vi "PicoScope4000aExampleBlock.vi"() -> ()   [LabVIEW 2010]
doc: "This example demonstrates how to use the PicoScope Labview library to collect data using block mode."
uses:
  shared/PicoBuffers.ctl
  shared/Buffer and Transfer Settings.ctl
  shared/Acquisition Settings.ctl
  PicoScope4000aLib/PicoScope4000aAnalogChannelSettings.ctl
panel:
  in  "roundFaster":bool=TRUE
  in  "Write to TDMS":bool
  in  "Channel B Settings":T1={"Enabled"=FALSE, "Coupling"=1, "Range"=6, "Analogue Offset"=0.0, "Bandwidth Limit"=0} {"Bandwidth Limit" items=["Full", "20kHz", "100kHz", "1MHz"]; "Range" items=["10 mV", "20 mV", "50 mV", "100 mV", "200 mV", "500 mV", "1 V", "2 V", "5 V", "10 V", "20 V", "50 V ", "100 V"]; "Coupling" items=["AC", "DC"]}
  in  "timeIntervalRequested":dbl format="%#6_6p"
  out "Pico 4000a Units":string
  out "Unit Info":T2
  in  "Resolution":u32(ring)=1 items=["8-bit", "12-bit", "14-bit"]
  in  "Trigger Settings":T3={"Trigger Enabled"=FALSE, "Trigger Source"=enum."Channel A", "Trigger Threshold (Volts/Probe units)"=0.0, "Trigger Direction"=2, "Trigger Delay (samples)"=0, "Auto Trigger Time (ms)"=1000} {"Trigger Direction" items=["Rising"=2, "Falling"=3]}
  out "overflow":i16 format="%08b"
  in  "Apply Settings":bool
  in  "Channel A Settings":T1={"Enabled"=TRUE, "Coupling"=1, "Range"=8, "Analogue Offset"=0.0, "Bandwidth Limit"=0} {"Bandwidth Limit" items=["Full", "20kHz", "100kHz", "1MHz"]; "Range" items=["10 mV", "20 mV", "50 mV", "100 mV", "200 mV", "500 mV", "1 V", "2 V", "5 V", "10 V", "20 V", "50 V ", "100 V"]; "Coupling" items=["AC", "DC"]}
  out "USB 3.0 device on non-USB 3.0 Port":bool=TRUE
  out "USB Powered":bool=TRUE
  out "error out":errorcluster
  in  "Data file":path=path "PicoScope4000aExampleBlock"
  in  "Buffer and Transfer Settings":T4={"startIndex"=0, "Samples"=1000000, "Down Sample Ratio"=1, "Down-Sample Mode"=0} {"Down-Sample Mode" items=["RAW none"=2147483648, "None"=0, "Aggregate"=1, "Decimate"=2, "Average"=4]; "Down Sample Ratio" step=1; "Samples" format="%_6p"}
  in  "Acquisition Settings":T5={"preTriggerSamples"=0, "postTriggerSamples"=1000000, "timebase"=0} {"postTriggerSamples" format="%_6p"; "preTriggerSamples" format="%_6p"}
  out "Properties Panel":T6 {"Max Total Capture Time Available (sec)" format="%.3p"; "Sample Frequency" format="%.6p"; "Sample Rate" format="%.3p"; "Max Samples Available" format="%_6p"; "Total Capture Time (sec)" format="%.3p"}
  in  "stop":bool
  out "Analog Channels":cluster{i32, dbl, "Data":dbl[]}[](graph)
  in  "Serial Number":string
  in  "Use Serial Number":bool
  in  "error in (no error)":errorcluster
  # "Bit 0 = ChA"
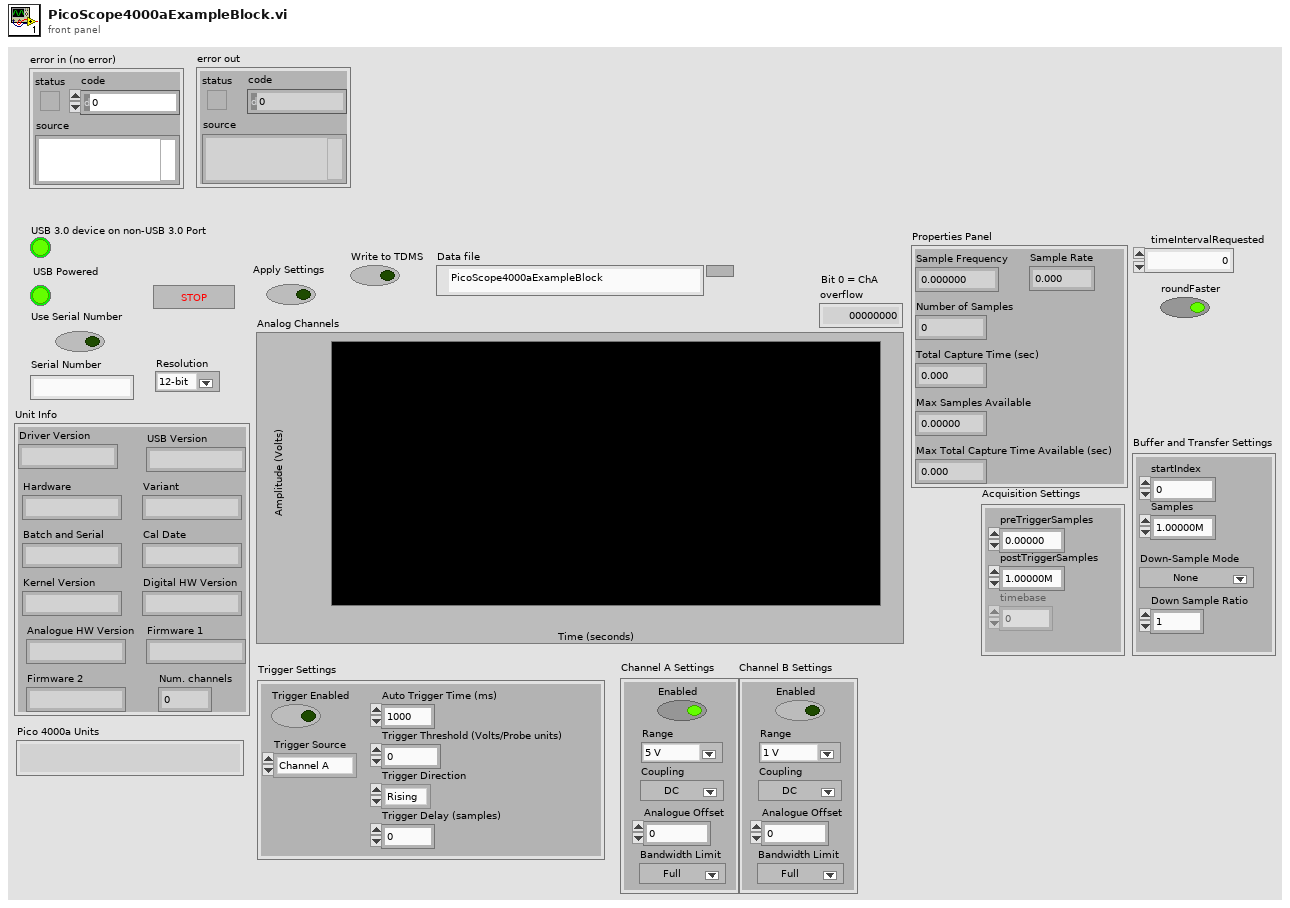
[diagram p1: front panel]
types:
  T1 = typedef "PicoScope4000aAnalogChannelSettings.ctl" = cluster{"Enabled":bool, "Coupling":i16, "Range":u32, "Analogue Offset":sgl, "Bandwidth Limit":u32}
  T2 = cluster{"Driver Version":string, "USB Version":string, "Hardware":string, "Variant":string, "Batch and Serial":string, "Cal Date":string, "Kernel Version":string, "Digital HW Version":string, "Analogue HW Version":string, "Firmware 1":string, "Firmware 2":string, "Num. channels":i16}
  T3 = cluster{"Trigger Enabled":bool, "Trigger Source":enum16{"Channel A", "Channel B", "Channel C", "Channel D", "Channel E", "Channel F", "Channel G", "Channel H"}, "Trigger Threshold (Volts/Probe units)":dbl, "Trigger Direction":u16, "Trigger Delay (samples)":u32, "Auto Trigger Time (ms)":i16}
  T4 = typedef "Buffer and Transfer Settings.ctl" = cluster{"startIndex":u64, "Samples":u64, "Down Sample Ratio":u64, "Down-Sample Mode":u32}
  T5 = typedef "Acquisition Settings.ctl" = cluster{"preTriggerSamples":u64, "postTriggerSamples":u64, "timebase":u32}
  T6 = cluster{"Sample Frequency":dbl, "Sample Rate":dbl, "Max Samples Available":u64, "Number of Samples":u64, "Total Capture Time (sec) ":dbl, "Max Total Capture Time Available (sec)":dbl}
  T7 = typedef "PicoBuffers.ctl" = cluster{"Max Buffer Pointers":u64[][][], "Min Buffer Pointers":u64[][][], "StreamingDataInfo":cluster{"Channel":u32, "Down-Sample Mode":u32, "PICO_DATA_TYPE":enum32{"PICO_INT8_T", "PICO_INT16_T", "PICO_INT32_T", "PICO_UINT32_T", "PICO_INT64_T", ""}, "Samples":i32, "bufferIndex":u64, "startIndex":i32, "overflow":i16}[][]}
  T8 = enum16{"open", "open or create", "create or replace", "create", "open (read-only)"}
  T9 = cluster{"Channel A Buffer":i16[], "Channel B Buffer":i16[], "Channel C Buffer":i16[], "Channel D Buffer":i16[], "Channel E Buffer":i16[], "Channel F Buffer":i16[], "Channel G Buffer":i16[], "Channel H Buffer":i16[], "Port 0 Buffer":i16[], "Port 1 Buffer":i16[]}[]
  T10 = cluster{"Channel A Buffer":i16[], "Channel B Buffer":i16[], "Channel C Buffer":i16[], "Channel D Buffer":i16[], "Channel E Buffer":i16[], "Channel F Buffer":i16[], "Channel G Buffer":i16[], "Channel H Buffer":i16[], "Port 0 Buffer":i16[], "Port 1 Buffer":i16[]}
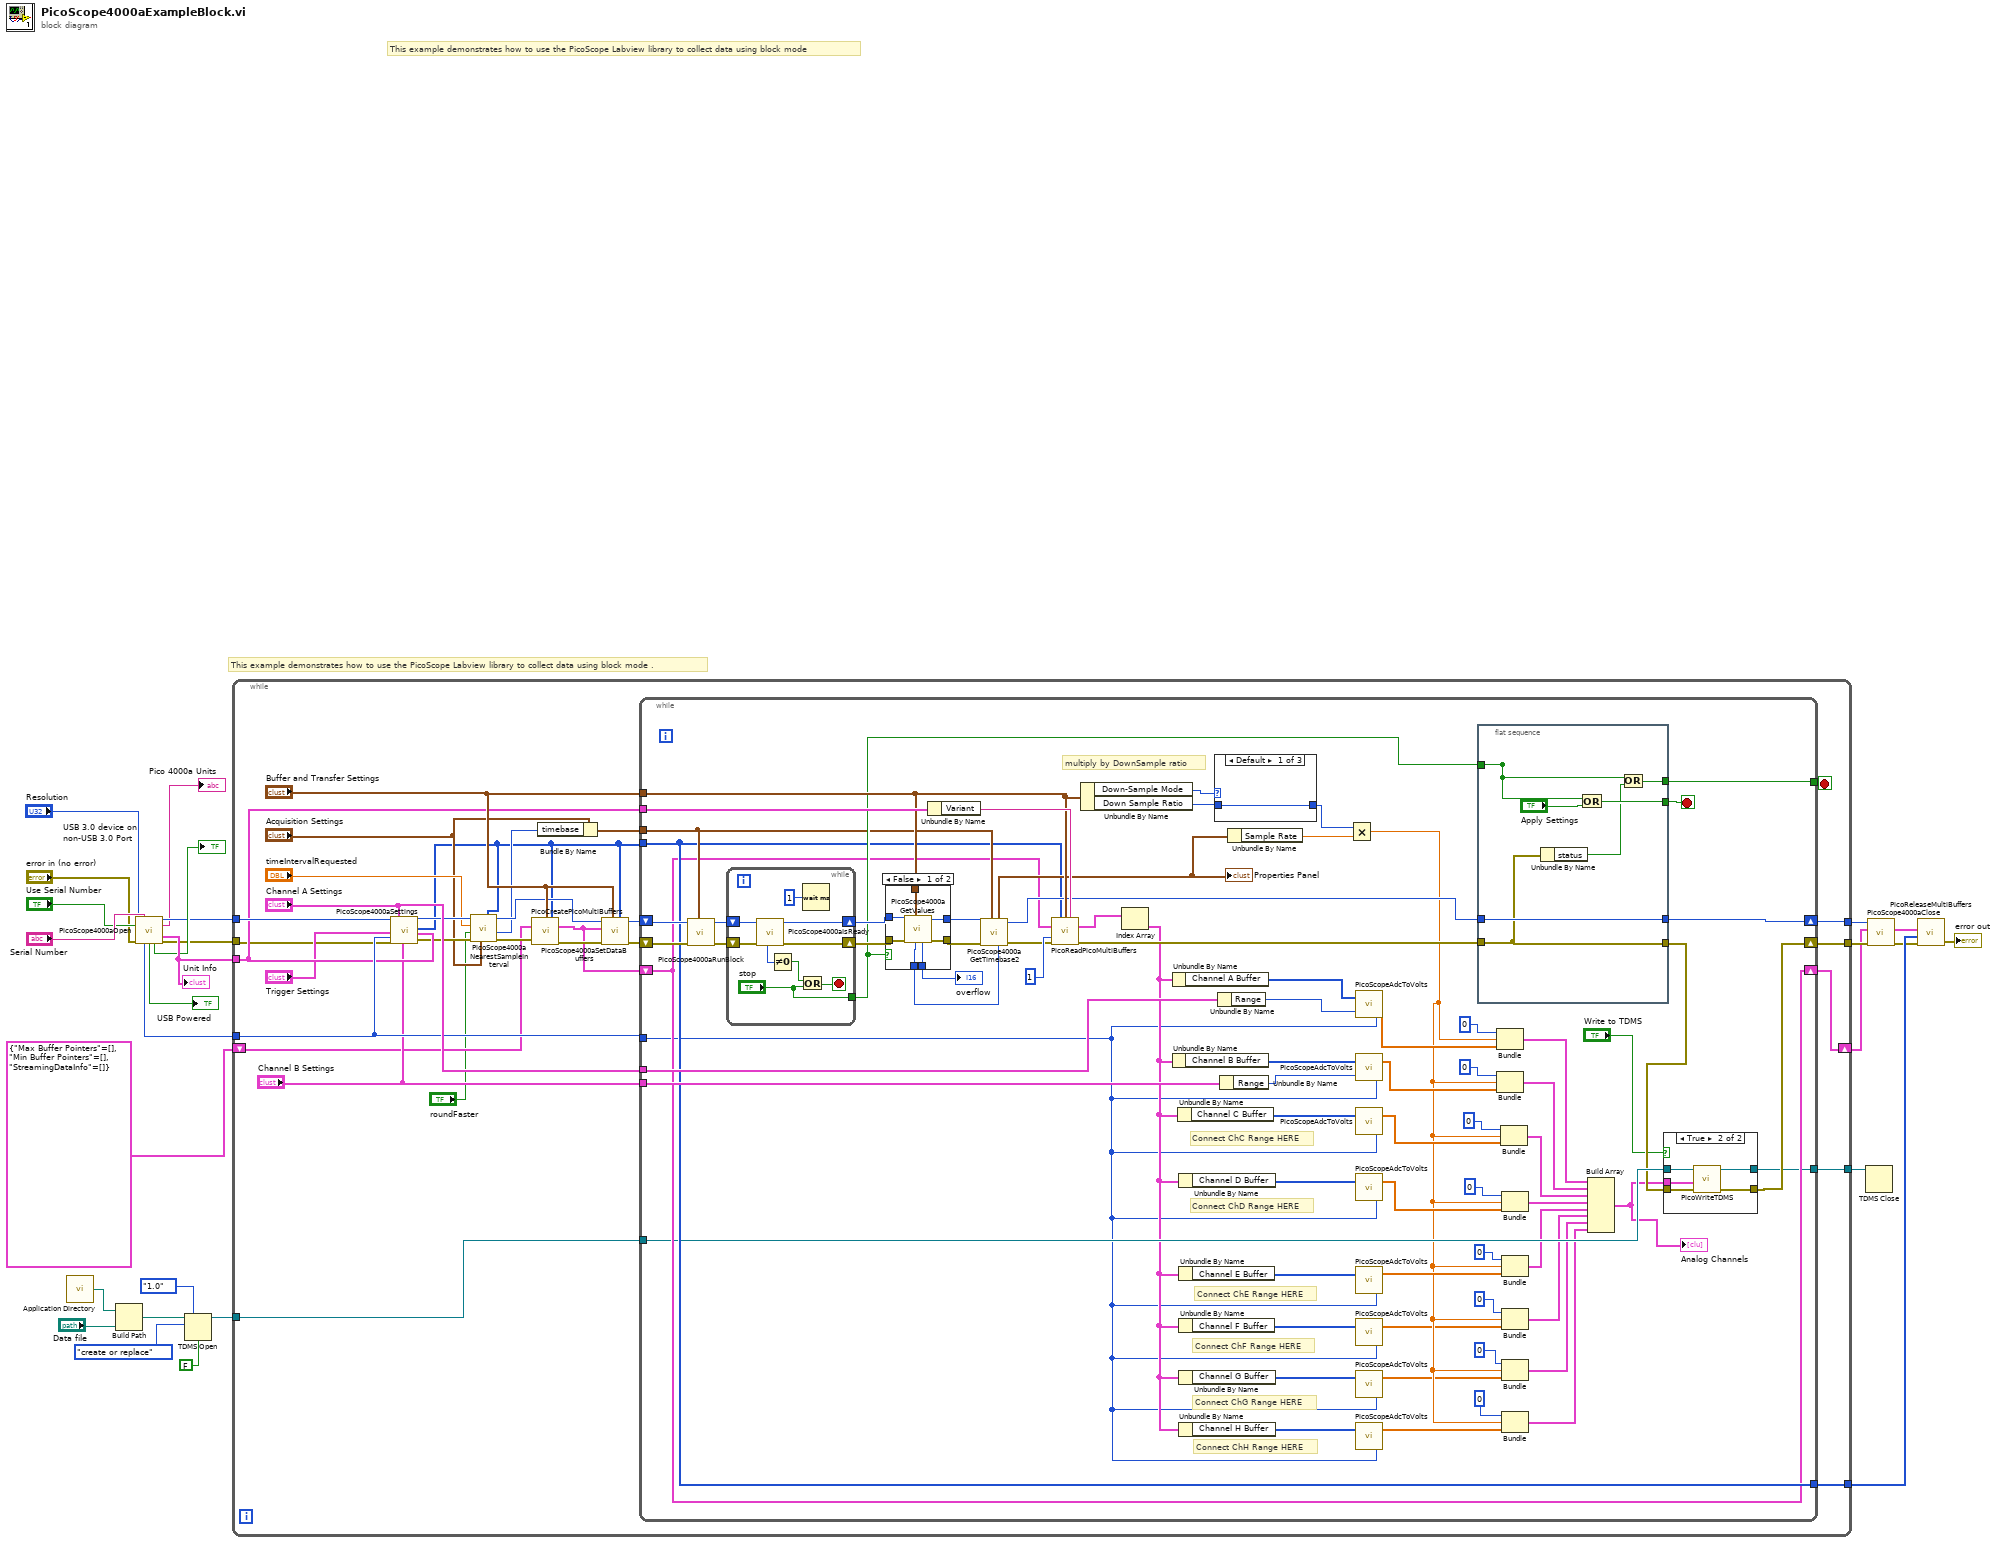
[diagram p0: block diagram]
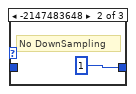
[diagram p4: hidden frame]
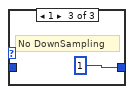
[diagram p5: hidden frame]
diagram:
  # "This example demonstrates how to use the PicoScope Labview library to collect data using block mode ."
  # "This example demonstrates how to use the PicoScope Labview library to collect data using block mode"
  n1 = call <vilib>:"Application Directory.vi"() -> ("Application Directory"=w20:path)
  n2 = Build Path(base path=w20, name or relative path="Data file") -> (appended path=w21:path)
  n3 = call "PicoScope4000aOpen.vi"("Serial Number"="Serial Number", "Use Serial Number"="Use Serial Number", "Resolution"="Resolution", "error in (no error)"="error in (no error)") -> ("handle"=w12:i16, "Pico 4000a Units"=→"Pico 4000a Units":string, "Unit Info"=w15:T2, "Max ADC value"=w16:i16, "USB powered"=→"USB Powered":bool, "USB 3.0 on non-USB 3.0 port"=→"USB 3.0 device on non-USB 3.0 Port":bool, "error out"=w6:errorcluster)  [unwired: 4 in, 1 out]
  "Unit Info" <- w15
  n4 = TDMS Open(6:FALSE ("disable buffering? (T)"), 7:enum16{"1.0", "2.0"}."1.0" ("file format version (2.0)"), 10:T8."create or replace" ("operation (0:open)"), 11:w21) -> (3:w18:refnum<k34>)  [unwired: 2 in, 1 out]
  n5 = while {
    tunnel: w6 -> [w41]
    tunnel: w16 -> [w51]
    tunnel: [w31] -> w26
    tunnel: [w49] -> w19
    tunnel: w18 -> [w54]
    tunnel: w12 -> [w53]
    tunnel: [w50] -> w9
    tunnel: [w47] -> w7
    tunnel: w15 -> [w43]
    shift-right: [w30] -> w1
    shift-left: T7 {"Max Buffer Pointers"=[], "Min Buffer Pointers"=[], "StreamingDataInfo"=[]} ("Data Pointers") -> [w29]
    stop <- w48 stop-if-true
    n6 = call "PicoScope4000aSettings.vi"("handle in"=w53, "Trigger Settings"="Trigger Settings", "Max ADC value"=w51, "error in"=w41, "Channel A Settings"="Channel A Settings", "Channel B Settings"="Channel B Settings", "Unit Info"=w43) -> ("handle out"=w37:i16, "Enabled array"=w27:i16[], "error out"=w40:errorcluster)  [unwired: 10 in]
    n7 = call "PicoScope4000aNearestSampleInterval.vi"("Enabled array"=w27, "Acquisition Settings"="Acquisition Settings", "error in (no error)"=w40, "roundFaster"="roundFaster", "timeIntervalRequested"="timeIntervalRequested", "handle in"=w37) -> ("error out"=w39:errorcluster, "timebase"=w33:u32, "handle out"=w38:i16)  [unwired: 2 in, 1 out]
    n8 = call "PicoCreatePicoMultiBuffers.vi"("Buffer and Transfer Settings"="Buffer and Transfer Settings", "enabled array"=w27, "Data Pointers In"=w29, "error in (no error)"=w39) -> ("Data Pointers"=w55:T7, "error out"=w56:errorcluster)  [unwired: 10 in]
    n9 = Bundle By Name(cluster="Acquisition Settings", "timebase"=w33) -> (w35:T5)
    n10 = call "PicoScope4000aSetDataBuffers.vi"("enabled array"=w27, "Buffer and Transfer Settings"="Buffer and Transfer Settings", "error in (no error)"=w56, "Data Pointers In"=w55, "handle in"=w38) -> ("error out"=w46:errorcluster, "handle out"=w45:i16)  [unwired: 5 in]
    n11 = while {
      tunnel: "Buffer and Transfer Settings" -> [w95]
      tunnel: w27 -> [w83]
      tunnel: "Channel A Settings" -> [w125]
      tunnel: w35 -> [w86]
      tunnel: w51 -> [w71]
      tunnel: w43 -> [w122]
      tunnel: [w102] -> w48
      shift-right: [w79] -> w50
      shift-left: w46 -> [w96]
      shift-right: [w100] -> w47
      shift-left: w45 -> [w97]
      tunnel: w54 -> [w81]
      tunnel: [w78] -> w49
      tunnel: "Channel B Settings" -> [w84]
      tunnel: [w83] -> w31
      shift-right: [w82] -> w30
      shift-left: w55 -> [w82]
      stop <- w101 stop-if-true
      # "Connect ChF Range HERE"
      # "Connect ChE Range HERE"
      # "Connect ChH Range HERE"
      # "Connect ChG Range HERE"
      # "Connect ChD Range HERE"
      # "Connect ChC Range HERE"
      # "multiply by DownSample ratio"
      n12 = call "PicoScope4000aRunBlock.vi"("Acquisition Settings"=w86, "error in (no error)"=w96, "handle in"=w97) -> ("error out"=w127:errorcluster, "handle out"=w126:i16)  [unwired: 5 in, 2 out]
      n13 = while {
        shift-right: [w162] -> w98
        shift-left: w127 -> [w163]
        shift-right: [w161] -> w99
        shift-left: w126 -> [w160]
        tunnel: ["stop"] -> w94
        stop <- w157 stop-if-true
        n14 = call "PicoScope4000aIsReady.vi"("error in (no error)"=w163, "handle in"=w160) -> ("error out"=w162:errorcluster, "handle out"=w161:i16, "ready"=w159:i16)  [unwired: 7 in]
        n15 = Not Equal To 0?(x=w159) -> (x != 0?=w158:bool)
        n16 = Or(x=w158, y="stop") -> (x .or. y?=w157:bool)
        n17 = Wait (ms)(milliseconds to wait=u32 1) -> ()  [unwired: 1 out]
      }
      n18 = case shown="False" w94 {
        tunnel: w98 -> [w145 w146]
        tunnel: w99 -> [w144 w147]
        tunnel: [w143 w147] -> w88
        tunnel: [w142 w146] -> w89
        tunnel: w95 -> [w141 _]
        tunnel: [w140 _] -> w93
        tunnel: [w139 _] -> w92
        frame False {
          n19 = call "PicoScope4000aGetValues.vi"("Buffer and Transfer Settings"=w141, "error in (no error)"=w145, "handle in"=w144) -> ("error out"=w142:errorcluster, "handle out"=w143:i16, "overflow"=w140:i16, "noOfSamples"=w139:u64)  [unwired: 5 in]
        }
        frame True {
        }
      }
      "overflow" <- w93
      n20 = Unbundle By Name(w122) -> ("Variant"=w123:string)
      n21 = call "PicoScope4000aGetTimebase2.vi"("Number of Samples"=w92, "Acquisition Settings"=w86, "error in (no error)"=w89, "handle in"=w88) -> ("error out"=w90:errorcluster, "handle out"=w87:i16, "Properties Panel"=w91:T6)  [unwired: 5 in]
      "Properties Panel" <- w91
      n22 = call "PicoReadPicoMultiBuffers.vi"("enabled array"=w83, "Buffer and Transfer Settings"=w95, "Variant"=w123, "Data Pointers"=w82, "No of Buffers"=1, "error in (no error)"=w90) -> ("MultiBuffers (Max or non-aggregated)"=w131:T9, "error out"=w103:errorcluster)  [unwired: 7 in, 1 out]
      n23 = Unbundle By Name(w95) -> ("Down-Sample Mode"=w129:u32, "Down Sample Ratio"=w130:u64)
      n24 = Index Array(array=w131) -> (element=w72:T10)  [unwired: 1 in]
      n25 = Unbundle By Name(w72) -> ("Channel A Buffer"=w112:i16[])
      n26 = Unbundle By Name(w72) -> ("Channel B Buffer"=w117:i16[])
      n27 = Unbundle By Name(w72) -> ("Channel C Buffer"=w110:i16[])
      n28 = Unbundle By Name(w72) -> ("Channel D Buffer"=w106:i16[])
      n29 = Unbundle By Name(w72) -> ("Channel G Buffer"=w75:i16[])
      n30 = Unbundle By Name(w72) -> ("Channel H Buffer"=w74:i16[])
      n31 = Unbundle By Name(w72) -> ("Channel E Buffer"=w73:i16[])
      n32 = Unbundle By Name(w72) -> ("Channel F Buffer"=w76:i16[])
      n33 = case shown="Default" w129 {
        tunnel: [w164 u64 1 ("Down Sample Ratio") u64 1 ("Down Sample Ratio")] -> w128
        tunnel: w130 -> [w164 _ _]
        frame Default {
        }
        frame -2147483648 {
          # "No DownSampling"
        }
        frame 1 {
          # "No DownSampling"
        }
      }
      n34 = Unbundle By Name(w125) -> ("Range"=w119:u32)
      n35 = Unbundle By Name(w84) -> ("Range"=w85:u32)
      n36 = Unbundle By Name(w91) -> ("Sample Rate"=w124:dbl)
      n37 = Multiply(x=w128, y=w124) -> (x*y=w65:dbl)
      n38 = call "PicoScopeAdcToVolts.vi"("Max_adc"=w71, "Range Index"=w119, "Data"=w112) -> ("Data"=w113:dbl[])
      n39 = call "PicoScopeAdcToVolts.vi"("Max_adc"=w71, "Range Index"=w85, "Data"=w117) -> ("Data"=w116:dbl[])
      n40 = call "PicoScopeAdcToVolts.vi"("Max_adc"=w71, "Data"=w110) -> ("Data"=w109:dbl[])  [unwired: 1 in]
      n41 = call "PicoScopeAdcToVolts.vi"("Max_adc"=w71, "Data"=w106) -> ("Data"=w105:dbl[])  [unwired: 1 in]
      n42 = call "PicoScopeAdcToVolts.vi"("Max_adc"=w71, "Data"=w73) -> ("Data"=w70:dbl[])  [unwired: 1 in]
      n43 = call "PicoScopeAdcToVolts.vi"("Max_adc"=w71, "Data"=w76) -> ("Data"=w64:dbl[])  [unwired: 1 in]
      n44 = call "PicoScopeAdcToVolts.vi"("Max_adc"=w71, "Data"=w75) -> ("Data"=w63:dbl[])  [unwired: 1 in]
      n45 = call "PicoScopeAdcToVolts.vi"("Max_adc"=w71, "Data"=w74) -> ("Data"=w62:dbl[])  [unwired: 1 in]
      n46 = flat-sequence {
        tunnel: [w154] -> w101
        tunnel: [w148] -> _
        tunnel: [w151] -> w102
        tunnel: w87 -> [w150]
        tunnel: [w150] -> w100
        tunnel: w103 -> [w149]
        tunnel: [w149] -> w80
        tunnel: w94 -> [w148]
        frame #0 {
          n47 = Unbundle By Name(w149) -> ("status"=w152:bool)
          n48 = Or(x=w148, y="Apply Settings") -> (x .or. y?=w154:bool)
          n49 = Or(x=w148, y=w152) -> (x .or. y?=w151:bool)
        }
      }
      n50 = Bundle(0, w65, "Data"=w113) -> (w115:cluster{i32, dbl, "Data":dbl[]})  [unwired: 1 in]
      n51 = Bundle(0, w65, "Data"=w116) -> (w114:cluster{i32, dbl, "Data":dbl[]})  [unwired: 1 in]
      n52 = Bundle(0, w65, "Data"=w109) -> (w108:cluster{i32, dbl, "Data":dbl[]})  [unwired: 1 in]
      n53 = Bundle(0, w65, "Data"=w105) -> (w104:cluster{i32, dbl, "Data":dbl[]})  [unwired: 1 in]
      n54 = Bundle(0, w65, "Data"=w70) -> (w60:cluster{i32, dbl, "Data":dbl[]})  [unwired: 1 in]
      n55 = Bundle(0, w65, "Data"=w64) -> (w59:cluster{i32, dbl, "Data":dbl[]})  [unwired: 1 in]
      n56 = Bundle(0, w65, "Data"=w63) -> (w58:cluster{i32, dbl, "Data":dbl[]})  [unwired: 1 in]
      n57 = Bundle(0, w65, "Data"=w62) -> (w57:cluster{i32, dbl, "Data":dbl[]})  [unwired: 1 in]
      n58 = Build Array(w115, w114, w108, w104, w60, w59, w58, w57) -> (w61:cluster{i32, dbl, "Data":dbl[]}[])
      "Analog Channels" <- w61
      n59 = case shown="True" "Write to TDMS" {
        tunnel: w61 -> [_ w138]
        tunnel: w81 -> [w132 w137]
        tunnel: w80 -> [w133 w136]
        tunnel: [w133 w135] -> w79
        tunnel: [w132 w134] -> w78
        frame False {
        }
        frame True {
          n60 = call "PicoWriteTDMS.vi"("error in (no error)"=w136, "Analog Channels"=w138, "Refnum in"=w137) -> ("error out"=w135:errorcluster, "Refnum out"=w134:refnum<k34>)  [unwired: 7 in]
        }
      }
    }
  }
  n61 = TDMS Close(11:w19) -> ()  [unwired: 1 in, 2 out]
  n62 = call "PicoScope4000aClose.vi"("error in (no error)"=w9, "handle in"=w7) -> ("error out"=w8:errorcluster)  [unwired: 7 in, 1 out]
  n63 = call "PicoReleaseMultiBuffers.vi"("error in (no error)"=w8, "Enabled array"=w26, "Data Pointers"=w1) -> ("error out"=→"error out":errorcluster)  [unwired: 7 in, 1 out]
